vi "Configure Session.vi"(8 "error in":errorcluster, 11 "Plugin in":refnum<class "Digital Output Handler.lvclass">) -> (0 "error out":errorcluster, 3 "Plugin out":refnum<class "Digital Output Handler.lvclass">)   [LabVIEW 2023, in "Digital Output Handler.lvlib" / "Digital Output Handler.lvclass"]
uses:
  Digital Output Handler.lvclass
  C:/Program Files/National Instruments/LabVIEW 2023/vi.lib/FlexLogger/SDK/PluginSDK.lvlibp/PEFClasses/SDK/Plugin/Plugin.lvclass
  Digital Output Handler.lvclass/Digital Output Handler.ctl
  <vilib>/FlexLogger/SDK/PluginSDK.lvlibp/PEFClasses/SDK/Channel/Data Type_v2.ctl
  <vilib>/FlexLogger/SDK/PluginSDK.lvlibp/PEFClasses/SDK/Setpoint Consumer Channel/Setpoint Consumer Channel.lvclass
  C:/Program Files/National Instruments/LabVIEW 2023/vi.lib/FlexLogger/SDK/PluginSDK.lvlibp/PEFClasses/SDK/Channel/Channel.lvclass
  <vilib>/FlexLogger/SDK/PluginSDK.lvlibp/PEFClasses/SDK/Producer Channel/Producer Channel.lvclass
  Digital Output Global.vi
  <vilib>/FlexLogger/SDK/PluginSDK.lvlibp/PEFClasses/SDK/Plugin/ParameterAccess/Read I32.vi
  <vilib>/FlexLogger/SDK/PluginSDK.lvlibp/PEFClasses/SDK/Derived Timing Producer Channel/Create Derived Time Producer Channel_v2.vi
  <vilib>/FlexLogger/SDK/PluginSDK.lvlibp/PEFClasses/SDK/Setpoint Consumer Channel/Create Setpoint Consumer Channel.vi
  <vilib>/FlexLogger/SDK/PluginSDK.lvlibp/PEFClasses/SDK/Channel/Channel.lvclass
  <vilib>/FlexLogger/SDK/PluginSDK.lvlibp
  <vilib>/FlexLogger/SDK/PluginSDK.lvlibp/PEFClasses/SDK/Plugin/Plugin.lvclass
  C:/Program Files/National Instruments/LabVIEW 2023/vi.lib/FlexLogger/SDK/PluginSDK.lvlibp/PEFClasses/SDK/Processing Element/Processing Element.lvclass
  C:/dev/niflexlogger-plugins/plugins/Digital Output Handler/source/Digital Output Handler/Digital Output Handler.lvclass
  <vilib>/FlexLogger/SDK/PluginSDK.lvlibp/PEFClasses/SDK/Derived Timing Producer Channel/Derived Timing Producer Channel.lvclass
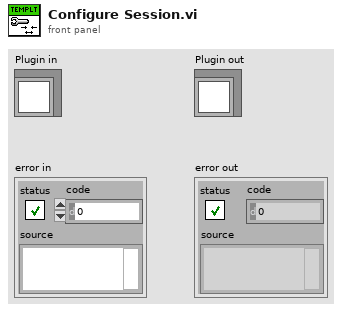
[diagram p1: front panel]
types:
  T1 = typedef "PluginSDK.lvlibp/Channel.lvclass/Data Type_v2.ctl" = u16
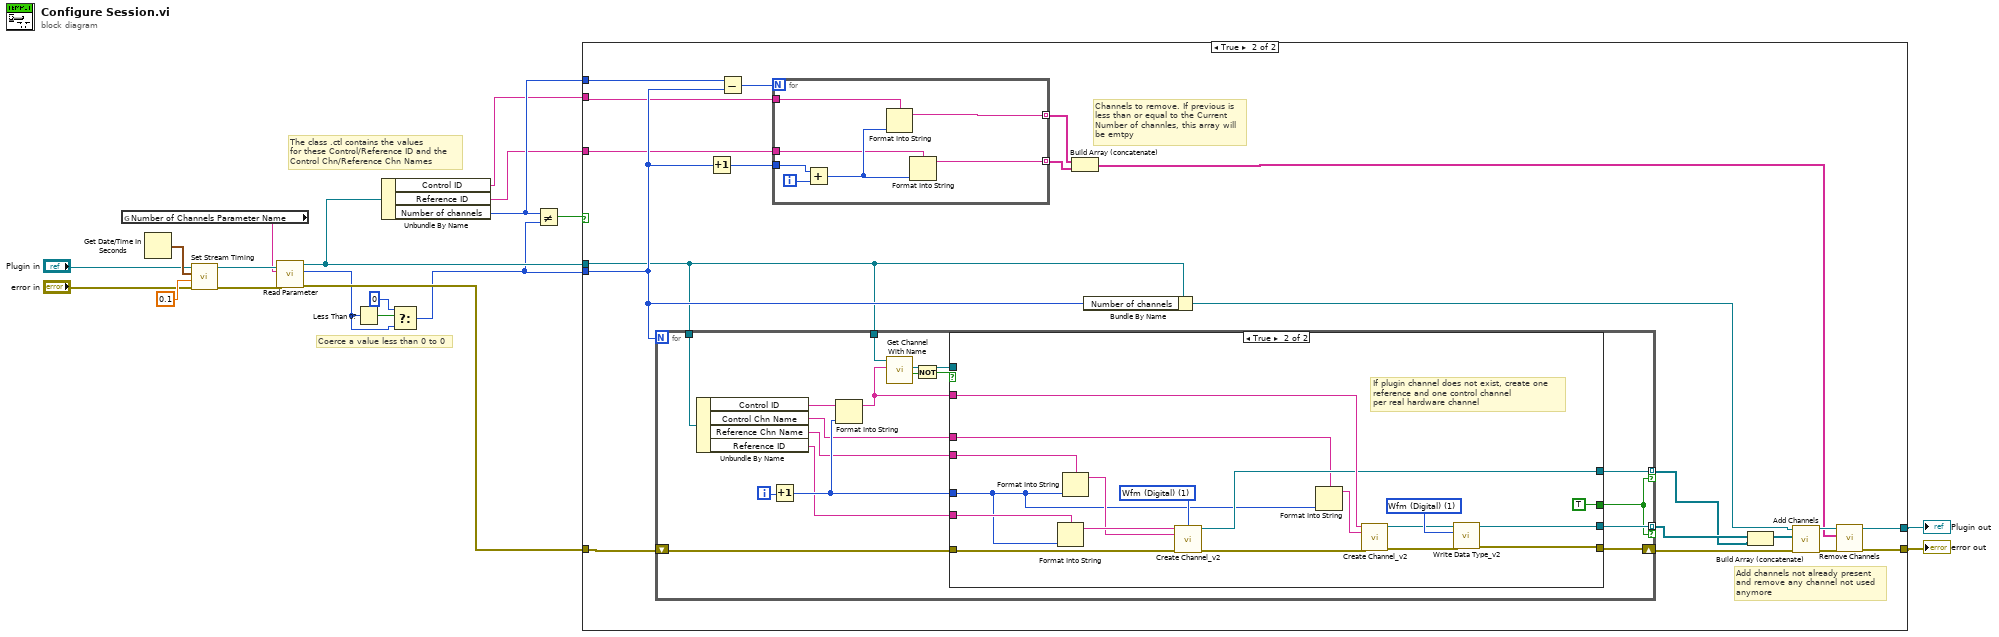
[diagram p0: block diagram]
diagram:
  # "Coerce a value less than 0 to 0"
  # "The class .ctl contains the values\nfor these Control/Reference ID and the\nControl Chn/Reference Chn Names"
  n1 = global read "Digital Output Global.vi" "Number of Channels Parameter Name"() -> (w1:string)
  n2 = Get Date/Time In Seconds() -> (seconds since 1Jan1904=w10:timestamp)
  n3 = call-dynamic "Set Stream Timing.vi"("error in (no error)"="error in", "dt(sec)"=0.1, "Start Time"=w10, "Plugin in"="Plugin in") -> ("error out"=w8:errorcluster, "Plugin out"=w7:refnum<class "Digital Output Handler.lvclass">)  [unwired: 6 in]
  n4 = call-poly <vilib>:"Read Parameter.vi"("error in (no error)"=w8, "Name"=w1, "Plugin in"=w7) -> ("error out"=w18:errorcluster, "Value"=w3:i32, "Plugin out"=w15:refnum<class "Digital Output Handler.lvclass">)  [unwired: 5 in, 1 out]
  n5 = Less Than 0?(x=w3) -> (x < 0?=w5:bool)
  n6 = Unbundle By Name(w15) -> ("Control ID"=w13:string, "Reference ID"=w12:string, "Number of channels"=w14:i32)
  n7 = Select(t=0, s=w5, f=w3) -> (s? t:f=w4:i32)
  n8 = Not Equal?(x=w14, y=w4) -> (x != y?=w19:bool)
  n9 = case shown="True" w19 {
    tunnel: w18 -> [w20 w41]
    tunnel: w15 -> [w21 w22]
    tunnel: w14 -> [_ w27]
    tunnel: w4 -> [_ w25]
    tunnel: [w21 w35] -> w17
    tunnel: [w20 w34] -> w16
    tunnel: w13 -> [_ w24]
    tunnel: w12 -> [_ w23]
    frame False {
    }
    frame True {
      # "Add channels not already present\nand remove any channel not used\nanymore"
      # "Channels to remove. If previous is less than or equal to the Current Number of channles, this array will be emtpy"
      n10 = for {
        N: w25 -> [_]
        tunnel: w22 -> [w58]
        tunnel: [w53] -> w37 mode=indexing if=w51
        tunnel: [w52] -> w38 mode=indexing if=w51
        shift-right: [w54] -> w36
        shift-left: w41 -> [w55]
        tunnel: w22 -> [w46]
        i -> [w50]
        n11 = Unbundle By Name(w46) -> ("Control ID"=w45:string, "Control Chn Name"=w43:string, "Reference Chn Name"=w44:string, "Reference ID"=w42:string)
        n12 = Increment(x=w50) -> (x+1=w48:i32)
        n13 = Format Into String(format string=w45, w48) -> (resulting string=w47:string)  [unwired: 2 in, 1 out]
        n14 = call <vilib>:"Get Channel With Name.vi"("Name"=w47, "Plugin in"=w58) -> ("Found?"=w57:bool, "Channel"=w49:refnum<class "Channel.lvclass">)  [unwired: 7 in, 1 out]
        n15 = Not(x=w57) -> (.not. x?=w56:bool)
        n16 = case shown="True" w56 {
          tunnel: w55 -> [w59 w75]
          tunnel: [_ w66] -> w52
          tunnel: [_ w69] -> w53
          tunnel: [w59 w67] -> w54
          tunnel: [_ TRUE] -> w51
          tunnel: w49 -> [_ _]
          tunnel: w48 -> [_ w60]
          tunnel: w47 -> [_ w71]
          tunnel: w44 -> [_ w63]
          tunnel: w43 -> [_ w62]
          tunnel: w42 -> [_ w61]
          frame False {
            # "If plugin channel is already present do nothing"
          }
          frame True {
            w68 = T1 1 items=["Wfm (DBL)", "Wfm (Digital)", "String"] ("Data Type")
            w76 = T1 1 items=["Wfm (DBL)", "Wfm (Digital)", "String"] ("Data Type")
            # "If plugin channel does not exist, create one\nreference and one control channel\nper real hardware channel"
            n17 = Format Into String(format string=w61, w60) -> (resulting string=w77:string)  [unwired: 2 in, 1 out]
            n18 = Format Into String(format string=w63, w60) -> (resulting string=w72:string)  [unwired: 2 in, 1 out]
            n19 = call-poly <vilib>:"Create Channel_v2.vi"("Unique Channel Identifier"=w77, "Data Type"=w76, "Default Channel Name"=w72, "error in (no error)"=w75) -> ("Producer Channel"=w69:refnum<class "Producer Channel.lvclass">, "error out"=w70:errorcluster)  [unwired: 10 in]
            n20 = Format Into String(format string=w62, w60) -> (resulting string=w73:string)  [unwired: 2 in, 1 out]
            n21 = call-poly <vilib>:"Create Channel_v2.vi"("Unique Channel Identifier"=w71, "Default Channel Name"=w73, "error in (no error)"=w70) -> ("Setpoint Consumer Channel"=w64:refnum<class "Setpoint Consumer Channel.lvclass">, "error out"=w65:errorcluster)  [unwired: 11 in]
            n22 = call-dynamic "Write Data Type_v2.vi"("error in (no error)"=w65, "Data Type"=w68, "Channel in"=w64) -> ("error out"=w67:errorcluster, "Channel out"=w66:refnum<class "Setpoint Consumer Channel.lvclass">)  [unwired: 7 in]
          }
        }
      }
      n23 = Increment(x=w25) -> (x+1=w26:i32)
      n24 = Subtract(x=w27, y=w25) -> (x-y=w28:i32)
      n25 = for {
        N: w28 -> [_]
        tunnel: [w84] -> w40 mode=indexing
        tunnel: [w83] -> w39 mode=indexing
        tunnel: w26 -> [w80]
        tunnel: w24 -> [w79]
        tunnel: w23 -> [w78]
        i -> [w82]
        n26 = Add(x=w80, y=w82) -> (x+y=w81:i32)
        n27 = Format Into String(format string=w79, w81) -> (resulting string=w84:string)  [unwired: 2 in, 1 out]
        n28 = Format Into String(format string=w78, w81) -> (resulting string=w83:string)  [unwired: 2 in, 1 out]
      }
      n29 = Build Array (concatenate)(w40, w39) -> (w29:string[])
      n30 = Bundle By Name(cluster=w22, "Number of channels"=w25) -> (w31:refnum<class "Digital Output Handler.lvclass">)
      n31 = Build Array (concatenate)(w38, w37) -> (w30:refnum<class "Channel.lvclass">[])
      n32 = call <vilib>:"Add Channels.vi"("error in (no error)"=w36, "Channels"=w30, "Plugin in"=w31) -> ("error out"=w33:errorcluster, "Plugin out"=w32:refnum<class "Digital Output Handler.lvclass">)  [unwired: 7 in]
      n33 = call-dynamic "Remove Channels.vi"("error in (no error)"=w33, "Unique Channel Identifiers to Delete"=w29, "Plugin in"=w32) -> ("error out"=w34:errorcluster, "Plugin out"=w35:refnum<class "Digital Output Handler.lvclass">)  [unwired: 7 in]
    }
  }
  "error out" <- w16
  "Plugin out" <- w17
